vi "Pin to Channel Name Extract.vi"(0 ".pinmap File Path":path, 2 "Pin Name":string) -> (7 "Channel":string)   [LabVIEW 2025, in "Digital Pattern Sequencer.lvclass"]
uses:
  Digital Pattern Sequencer.lvclass
  Digital Pattern Sequencer.lvclass/Digital Pattern Sequencer.ctl
  <resource>/objmgr/DOMUserDefRef.rc
  <vilib>/xml/NI_XML.lvlib
  <vilib>/xml/Load XML String.vi
  <vilib>/xml/XPath/Get All Matched Nodes (String).vi
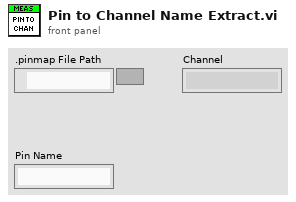
[diagram p1: front panel]
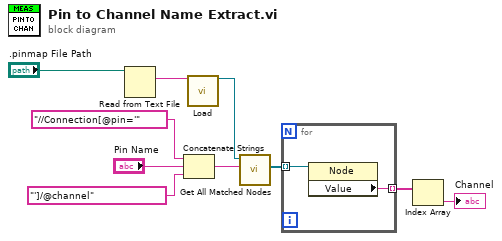
[diagram p0: block diagram]
diagram:
  n1 = Read from Text File(file (use dialog)=".pinmap File Path") -> (text=w8:string)  [unwired: 3 in, 3 out]
  n2 = Concatenate Strings("//Connection[@pin='" ("string"), "Pin Name", "']/@channel" ("string")) -> (w5:string)
  n3 = call-poly <vilib>:"Load.vi"("XML string"=w8) -> ("DOM document out"=w9:refnum<k20>)  [unwired: 12 in, 2 out]
  n4 = call-poly <vilib>:"Get All Matched Nodes.vi"("XPath expression"=w5, "node in"=w9) -> ("node result array"=w10:refnum<k20>[])  [unwired: 7 in, 2 out]
  n5 = for {
    tunnel: w10 -> [w12] mode=indexing
    tunnel: [w11] -> w4 mode=indexing
    n6 = property class="Node"(reference=w12) -> ("Value"=w11:string)  [unwired: 1 in, 2 out]
  }
  n7 = Index Array(array=w4) -> (element=→"Channel":string)  [unwired: 1 in]
